vi "Load Day.vi"(6 "Project Store in":refnum<class "Project Store.lvclass">, 7 "Time Entry Store in":refnum<class "Time Entry Store.lvclass">, 8 "error in":errorcluster, 10 "Now":timestamp, 11 "Day":timestamp) -> (0 "error out":errorcluster, 1 "Day Entries":T1, 2 "Row Entry IDs":string[](array[string]), 3 "Rows":string[][](array[string]), 4 "Project Store out":refnum<class "Project Store.lvclass">, 5 "Time Entry Store out":refnum<class "Time Entry Store.lvclass">)   [LabVIEW 2026]
doc: "Loads the time entries of one local calendar day for the TimeCard listbox. Calls the Time Entry Store's Read Entries for Day, sorts the entries by Start Time and formats each one with Format Entry Row.vi.\n\nInputs: Day (any time within the local day to show); Now (for the Elapsed column of a running entry); Time Entry Store in; Project Store in (for the project and task names); error in.\nOutputs: Rows (2D string, one row per entry - wire to the listbox Item Names); Row Entry IDs (entry ID of each row, same order); Day Entries (the entries, same order); Time Entry Store out; Project Store out; error out.\n\nGenerated by: Claude"
uses:
  Storage/Time Entry Store/Time Entry Store.lvclass
  Storage/Project Store/Project Store.lvclass
  Storage/Rows/Time Entry.ctl
  Storage/Rows/Time Entry List.ctl
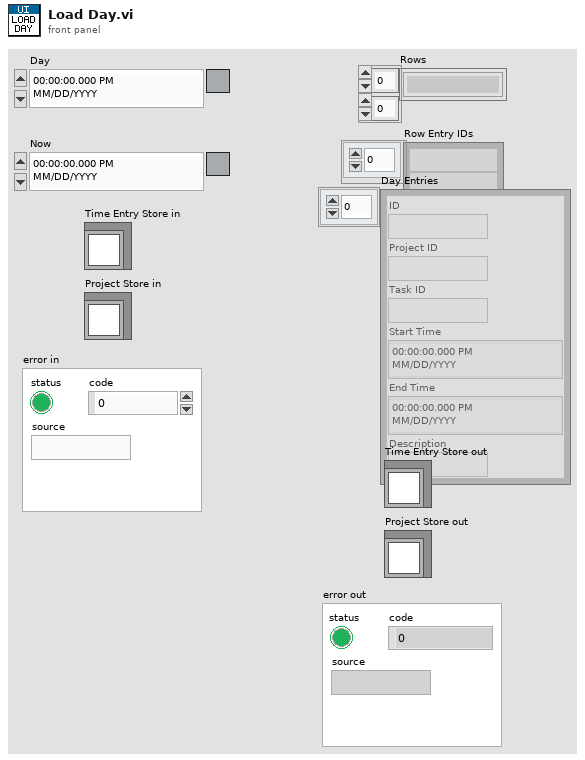
[diagram p1: front panel]
types:
  T1 = typedef "Time Entry List.ctl" = T2[]
  T2 = typedef "Time Entry.ctl" = cluster{"ID":string, "Project ID":string, "Task ID":string, "Start Time":timestamp, "End Time":timestamp, "Description":string}
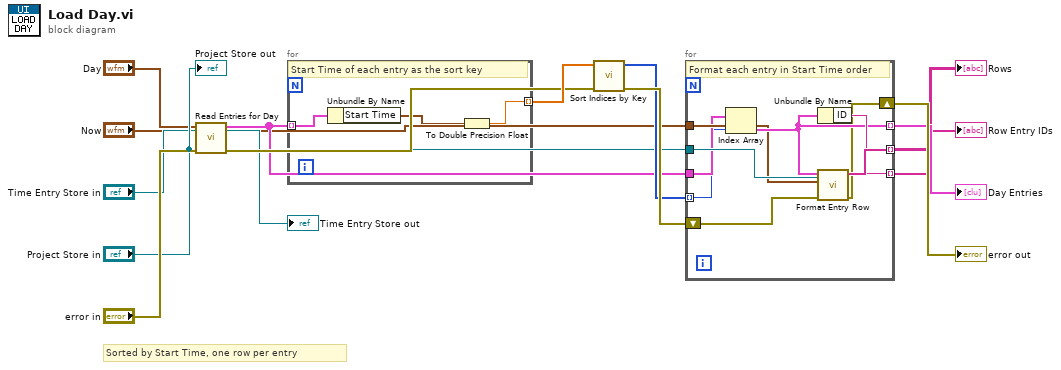
[diagram p0: block diagram]
diagram:
  # "Sorted by Start Time, one row per entry"
  n1 = call-dynamic "Read Entries for Day.vi"("Time Entry Store in"="Time Entry Store in", "error in (no error)"="error in", "Date"="Day") -> ("error out"=w12:errorcluster, "Time Entries"=w11:T1, "Time Entry Store out"=→"Time Entry Store out":refnum<class "Time Entry Store.lvclass">)  [unwired: 6 in]
  n2 = for {
    tunnel: w11 -> [w16] mode=indexing
    tunnel: [w18] -> w13 mode=indexing
    # "Start Time of each entry as the sort key"
    n3 = Unbundle By Name(w16) -> ("Start Time"=w17:timestamp)
    n4 = To Double Precision Float(number=w17) -> (double precision float=w18:dbl)
  }
  n5 = call "Sort Indices by Key.vi"("error in (no error)"=w12, "Keys"=w13) -> ("error out"=w15:errorcluster, "Sorted Indices"=w14:i32[])  [unwired: 8 in]
  n6 = for {
    tunnel: "Now" -> [w21]
    tunnel: "Project Store in" -> [w22]
    tunnel: w11 -> [w20]
    tunnel: w14 -> [w19] mode=indexing
    shift-right: [w24] -> w10
    shift-left: w15 -> [w23]
    tunnel: [w25] -> w8 mode=indexing
    tunnel: [w27] -> w6 mode=indexing
    tunnel: [w26] -> w7 mode=indexing
    # "Format each entry in Start Time order"
    n7 = Index Array(array=w20, index=w19) -> (element=w25:T2)
    n8 = Unbundle By Name(w25) -> ("ID"=w26:string)
    n9 = call "Format Entry Row.vi"("Project Store in"=w22, "error in"=w23, "Now"=w21, "Time Entry"=w25) -> ("error out"=w24:errorcluster, "Row"=w27:string[])  [unwired: 5 in, 1 out]
  }
  "Rows" <- w6
  "Row Entry IDs" <- w7
  "Day Entries" <- w8
  "error out" <- w10
  "Project Store out" <- "Project Store in"
